vi "Pt 1tache.vi"(3 "Indice tache":i8) -> (0 "Données Pt":string[](array[string]))   [LabVIEW 2022 SP3]
uses:
  Enum/Enum cdaq 1.ctl
  <vilib>/DAQmx/read.llb/DAQmx Read (Analog 2D DBL NChan NSamp).vi
  <vilib>/Analysis/baseanly.llb/Mean (DBL).vi
  Variables globales/Variable glob Pt.vi
  Variables globales/Variable glob generale.vi
  <vilib>/DAQmx/miscellaneous.llb/DAQmx Fill In Error Info.vi
  <resource>/objmgr/daqmx.rc
  <vilib>/Analysis/NI_AALBase.lvlib
panel:
  out "Sélection Pt":bool[](array[boolean])
  out "Nom tache Pt":refnum<k21>
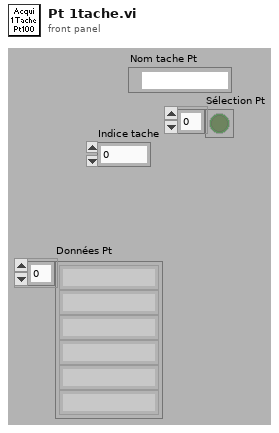
[diagram p1: front panel]
types:
  T1 = typedef "Enum cdaq 1.ctl" = enum16{"init", "acqui", "fin"}
  T2 = cluster{"Nom tache Pt":refnum<k21>, "Noms des Pt":string[], "Nb Pt":i16, "Selection Pt":bool[], "Nom Pt selectionnees":string[]}[]
  T3 = cluster{"Nom tache Pt":refnum<k21>, "Noms des Pt":string[], "Nb Pt":i16, "Selection Pt":bool[], "Nom Pt selectionnees":string[]}
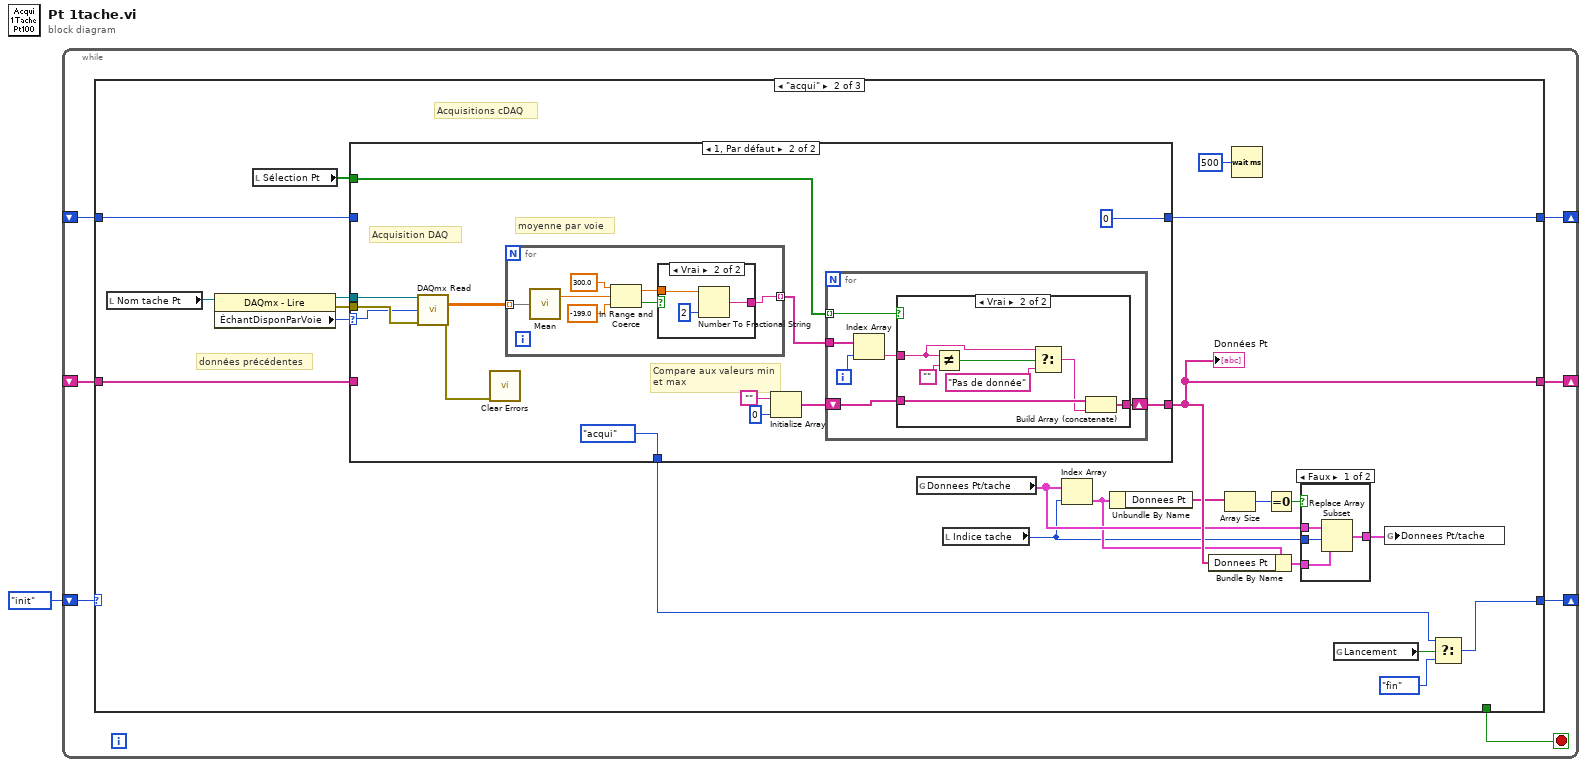
[diagram p0: block diagram]
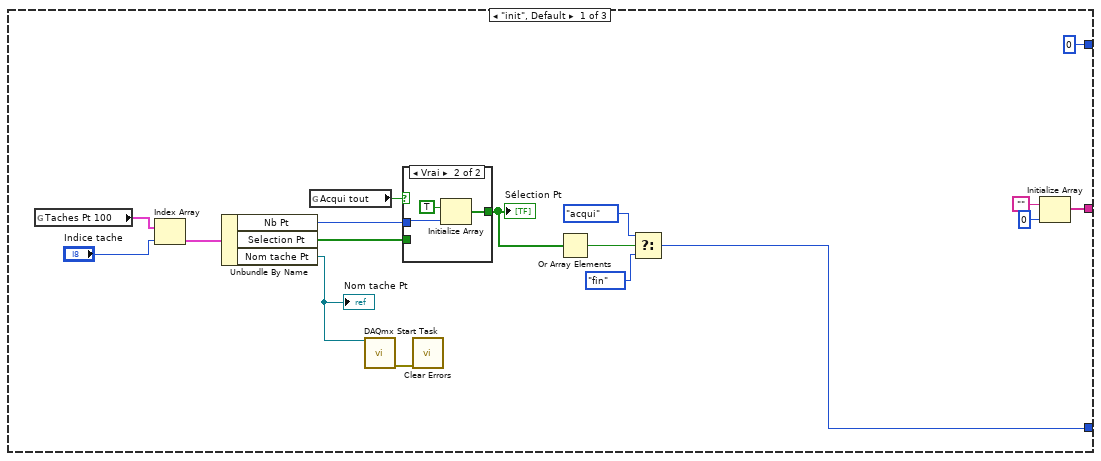
[diagram p2: hidden frame]
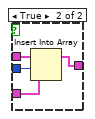
[diagram p4: hidden frame]
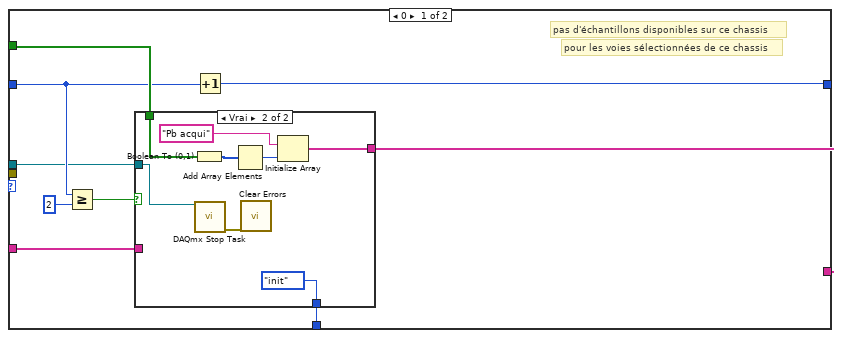
[diagram p5: hidden frame]
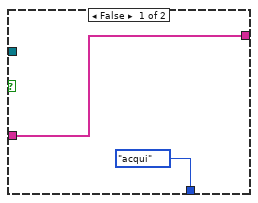
[diagram p6: hidden frame]
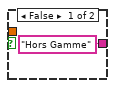
[diagram p8: hidden frame]
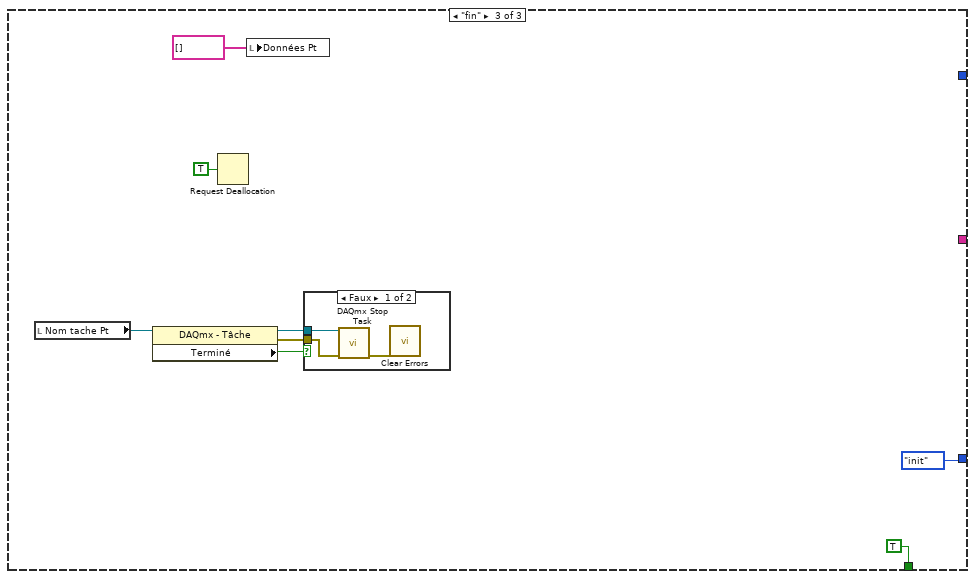
[diagram p9: hidden frame]
diagram:
  n1 = while {
    shift-right: [w7] -> _
    shift-left: Enum_cdaq_1."init" ("Énum") -> [w8]
    shift-right: [w5] -> _
    shift-left: _ -> [w6]
    shift-right: [w3] -> _
    shift-left: _ -> [w4]
    stop <- w2 stop-if-true
    n2 = case shown="\"acqui\"" w8 {
      tunnel: [w11 w45 Enum_cdaq_1."init" ("Énum")] -> w7
      tunnel: w6 -> [_ w51 _]
      tunnel: [0 w50 _] -> w5
      tunnel: w4 -> [_ w49 _]
      tunnel: [w13 w48 _] -> w3
      tunnel: [_ _ TRUE] -> w2
      frame "init", Default {
        n3 = global read "Variable glob Pt.vi" "Taches Pt 100"() -> (w23:T2)
        n4 = Index Array(array=w23, index="Indice tache") -> (element=w24:T3)
        n5 = Unbundle By Name(w24) -> ("Nb Pt"=w21:i16, "Selection Pt"=w20:bool[], "Nom tache Pt"=w9:refnum<k21>)
        "Nom tache Pt" <- w9
        n6 = global read "Variable glob generale.vi" "Acqui tout"() -> (w22:bool)
        n7 = call <vilib>:"DAQmx Start Task.vi"("task/channels in"=w9) -> ("error out"=w10:errorcluster)  [unwired: 13 in, 1 out]
        n8 = case shown="Vrai" w22 {
          tunnel: [w26 w28] -> w19
          tunnel: w20 -> [w26 _]
          tunnel: w21 -> [_ w27]
          frame False {
          }
          frame True {
            n9 = Initialize Array(TRUE, w27) -> (w28:bool[])
          }
        }
        "Sélection Pt" <- w19
        n10 = call <vilib>:"Clear Errors.vi"("error in (no error)"=w10) -> ()  [unwired: 5 in, 2 out]
        n11 = Or Array Elements(Boolean array=w19) -> (logical OR=w18:bool)
        n12 = Select(t=Enum_cdaq_1."acqui" ("Énum"), s=w18, f=Enum_cdaq_1."fin" ("Énum")) -> (s? t:f=w11:T1)
        n13 = Initialize Array("", 0 ("taille de la dimension")) -> (w13:string[])
      }
      frame "acqui" {
        # "données précédentes"
        # "Acquisitions cDAQ"
        n14 = local read "Nom tache Pt"() -> (w31:refnum<k21>)
        n15 = property class="DAQmx - Lire"(reference=w31) -> (reference out=w34:refnum<k21>, error out=w42:errorcluster, "ÉchantDisponParVoie"=w43:u32)  [unwired: 1 in]
        n16 = local read "Sélection Pt"() -> (w32:bool[])
        n17 = case shown="1, Par défaut" w43 {
          selector: w43 -> [_ w80]
          tunnel: [w68 w81] -> w48
          tunnel: w32 -> [w67 w83]
          tunnel: w34 -> [w60 w86]
          tunnel: w49 -> [w64 _]
          tunnel: w42 -> [_ w85]
          tunnel: [w66 0] -> w50
          tunnel: w51 -> [w65 _]
          tunnel: [w61 Enum_cdaq_1."acqui" ("Énum")] -> w30
          frame 0 {
            # "pour les voies sélectionnées de ce chassis"
            # "pas d'échantillons disponibles sur ce chassis"
            n18 = Greater Or Equal?(x=w65, y=2) -> (x >= y?=w62:bool)
            n19 = case shown="Vrai" w62 {
              tunnel: [w70 w74] -> w68
              tunnel: w67 -> [_ w77]
              tunnel: w64 -> [w70 _]
              tunnel: [Enum_cdaq_1."acqui" ("Énum") Enum_cdaq_1."init" ("Énum")] -> w61
              tunnel: w60 -> [_ w72]
              frame False {
              }
              frame True {
                n20 = Boolean To (0,1)(Boolean=w77) -> (0, 1=w76:i16[])
                n21 = call <vilib>:"DAQmx Stop Task.vi"("task/channels in"=w72) -> ("error out"=w71:errorcluster)  [unwired: 13 in, 1 out]
                n22 = Add Array Elements(numeric array=w76) -> (sum=w75:i16)
                n23 = call <vilib>:"Clear Errors.vi"("error in (no error)"=w71) -> ()  [unwired: 5 in, 2 out]
                n24 = Initialize Array("Pb acqui", w75) -> (w74:string[])
              }
            }
            n25 = Increment(x=w65) -> (x+1=w66:i32)
          }
          frame 1, Default {
            # "Acquisition DAQ"
            # "moyenne par voie"
            # "Compare aux valeurs min et max"
            n26 = call-poly <vilib>:"DAQmx Read.vi"("task/channels in"=w86, "number of samples per channel"=w80, "error in"=w85) -> ("data"=w90:dbl[][], "error out"=w84:errorcluster)  [unwired: 10 in, 1 out]
            n27 = call <vilib>:"Clear Errors.vi"("error in (no error)"=w84) -> ()  [unwired: 5 in, 2 out]
            n28 = for {
              tunnel: w90 -> [w112] mode=indexing
              tunnel: [w106] -> w91 mode=indexing
              n29 = call-poly <vilib>:"Mean.vi"("X"=w112) -> ("mean"=w109:dbl)  [unwired: 1 out]
              n30 = In Range and Coerce(upper limit=300.0 ("élément"), x=w109, lower limit=-199.0 ("élément")) -> (coerced(x)=w107:dbl, In Range?=w108:bool)
              n31 = case shown="Vrai" w108 {
                tunnel: w107 -> [_ w115]
                tunnel: ["Hors Gamme" w114] -> w106
                frame False {
                }
                frame True {
                  n32 = Number To Fractional String(number=w115, precision (6)=i16 2 ("précision (6)")) -> (F-format string=w114:string)  [unwired: 2 in]
                }
              }
            }
            n33 = Initialize Array("", 0 ("taille de la dimension")) -> (w89:string[])
            n34 = for {
              tunnel: w83 -> [w97] mode=indexing
              tunnel: w91 -> [w96]
              shift-right: [w92] -> w81
              shift-left: w89 -> [w93]
              i -> [w95]
              n35 = Index Array(array=w96, index=w95) -> (element=w94:string)
              n36 = case shown="Vrai" w97 {
                tunnel: w94 -> [_ w104]
                tunnel: w93 -> [w98 w102]
                tunnel: [w98 w101] -> w92
                frame False {
                  # "voie non sélectionnée"
                }
                frame True {
                  n37 = Not Equal?(x=w104, y="") -> (x != y?=w99:bool)
                  n38 = Select(t=w104, s=w99, f="Pas de donnée" ("cas faux")) -> (s? t:f=w100:string)
                  n39 = Build Array (concatenate)(w102, w100) -> (w101:string[])
                }
              }
            }
          }
        }
        "Données Pt" <- w48
        n40 = global read "Variable glob Pt.vi" "Donnees Pt/tache"() -> (w38:cluster{"Donnees Pt":string[]}[])
        n41 = local read "Indice tache"() -> (w33:i8)
        n42 = Index Array(array=w38, index=w33) -> (element=w37:cluster{"Donnees Pt":string[]})
        n43 = Unbundle By Name(w37) -> ("Donnees Pt"=w39:string[])
        n44 = Bundle By Name(cluster=w37, "Donnees Pt"=w48) -> (w36:cluster{"Donnees Pt":string[]})
        n45 = Array Size(array=w39) -> (size(s)=w40:i32)
        n46 = Wait (ms)(milliseconds to wait=u32 500 ("n millisecondes")) -> ()  [unwired: 1 out]
        n47 = Equal To 0?(x=w40) -> (x = 0?=w41:bool)
        n48 = case shown="Faux" w41 {
          tunnel: w36 -> [w55 w59]
          tunnel: [w54 w56] -> w35
          tunnel: w38 -> [w53 w58]
          tunnel: w33 -> [w52 w57]
          frame False {
            n49 = Replace Array Subset(array=w53, new element=w55, index=w52) -> (w54:cluster{"Donnees Pt":string[]}[])
          }
          frame True {
            n50 = Insert Into Array(array=w58, index=w57, new element=w59) -> (w56:cluster{"Donnees Pt":string[]}[])
          }
        }
        n51 = global read "Variable glob generale.vi" "Lancement"() -> (w47:bool)
        n52 = global write "Variable glob Pt.vi" "Donnees Pt/tache"(w35) -> ()
        n53 = Select(t=w30, s=w47, f=Enum_cdaq_1."fin" ("Énum")) -> (s? t:f=w45:T1)
      }
      frame "fin" {
        n54 = local read "Nom tache Pt"() -> (w119:refnum<k21>)
        n55 = property class="DAQmx - Tâche"(reference=w119) -> (reference out=w123:refnum<k21>, error out=w124:errorcluster, "Terminé"=w122:bool)  [unwired: 1 in]
        n56 = Request Deallocation(TRUE ("flag")) -> ()
        n57 = local write "Données Pt"(string[] [] ("Données Pt 1D")) -> ()
        n58 = case shown="Faux" w122 {
          tunnel: w123 -> [w127 _]
          tunnel: w124 -> [w126 _]
          frame False {
            n59 = call <vilib>:"DAQmx Stop Task.vi"("task/channels in"=w127, "error in"=w126) -> ("error out"=w125:errorcluster)  [unwired: 12 in, 1 out]
            n60 = call <vilib>:"Clear Errors.vi"("error in (no error)"=w125) -> ()  [unwired: 5 in, 2 out]
          }
          frame True {
          }
        }
      }
    }
  }
